vi "Pass++.vi"(9 "字符串":string="0", 10 "reset":bool) -> (1 "数值":u32)   [LabVIEW 2025]
uses:
  global.vi
  System.Windows.Forms
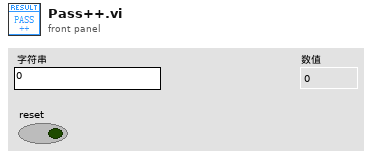
[diagram p1: front panel]
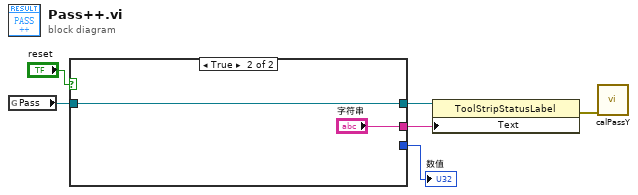
[diagram p0: block diagram]
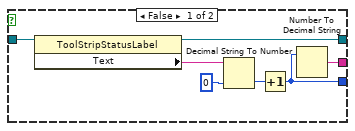
[diagram p2: hidden frame]
diagram:
  n1 = global read "global.vi" "Pass"() -> (w4:refnum<k24>)
  n2 = case shown="True" "reset" {
    tunnel: [w11 w15] -> w6
    tunnel: [w10 "字符串"] -> w5
    tunnel: w4 -> [w9 w15]
    tunnel: [w7 _] -> w1
    frame False {
      n3 = property class="ToolStripStatusLabel"(reference=w9) -> (reference out=w11:refnum<k24>, "Text"=w13:string)  [unwired: 1 in, 1 out]
      n4 = Decimal String To Number(string=w13, default (0L)=u32 0 ("默认(0 I32)")) -> (number=w12:u32)  [unwired: 2 out]
      n5 = Increment(x=w12) -> (x+1=w7:u32)
      n6 = Number To Decimal String(number=w7) -> (decimal integer string=w10:string)  [unwired: 1 out]
    }
    frame True {
    }
  }
  "数值" <- w1
  n7 = property class="ToolStripStatusLabel"(reference=w6, "Text"=w5) -> (error out=w2:errorcluster)  [unwired: 1 in, 1 out]
  n8 = call "calPassY.vi"("error in (no error)"=w2) -> ()  [unwired: 11 in]
